vi "Task Loop.vi"(8 "error in (no error)":errorcluster, 11 "ChartGuiTask in":refnum<class "ChartGuiTask.lvclass">) -> (0 "error out":errorcluster)   [LabVIEW 2020, in "VolatusDemo.lvlib" / "ChartGuiTask.lvclass"]
uses:
  ChartGuiTask.lvclass
  C:/dev/lv20CE/relink/lv-volatus/Volatus/Task/Task.lvclass
  ChartGuiTask.lvclass/ChartGuiTask.ctl
  Volatus/Task/Task.lvclass/Task.ctl
  Volatus/Event API/EventAPI.lvclass/EventAPI.ctl
  Volatus/EventHandler Messages/Handle Event Msg/Handle Event Msg.lvclass/Handle Event Msg.ctl
  <vilib>/ActorFramework/Message Enqueuer/Message Enqueuer.lvclass/Message Enqueuer.ctl
  Volatus/Event API/Report Event.vi
  Volatus/EventHandler Messages/Handle Event Msg/Send Handle Event.vi
  <vilib>/ActorFramework/Message Enqueuer/Enqueue.vi
  Volatus/EventHandler Messages/Handle Event Msg/Handle Event Msg.lvclass
  C:/Program Files (x86)/National Instruments/LabVIEW 2020/vi.lib/ActorFramework/Message/Message.lvclass
  lv-vecto/Vecto/Group/Group.lvclass
  C:/dev/lv20CE/relink/lv-vecto/Vecto/GroupAbstract/GroupAbstract.lvclass
  <vilib>/ActorFramework/Message Priority Queue/Priority Enqueue.vi
  Volatus/Task/Task.lvclass
  lv-vecto/Vecto/GroupAbstract/GroupAbstract.lvclass
panel:
  out "Chart":dbl[][](graph)
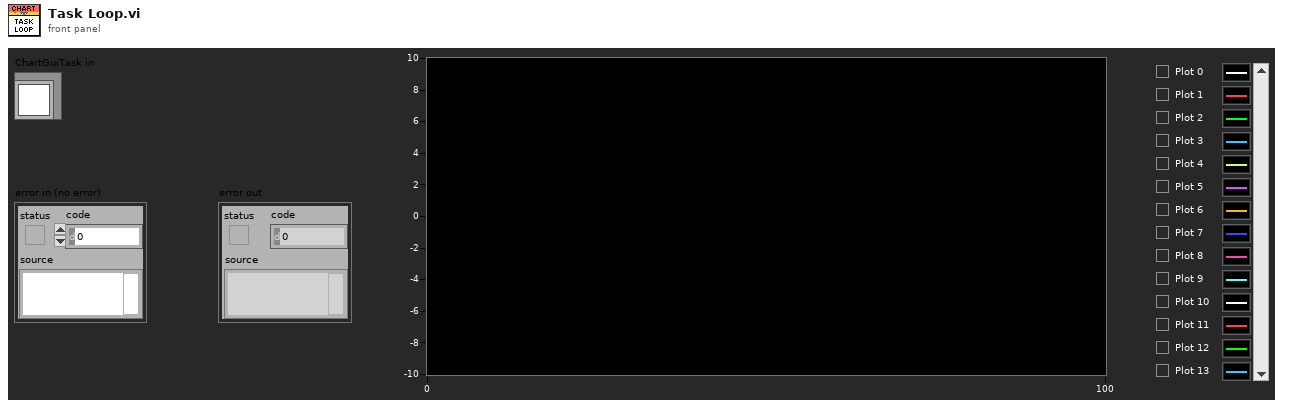
[diagram p1: front panel]
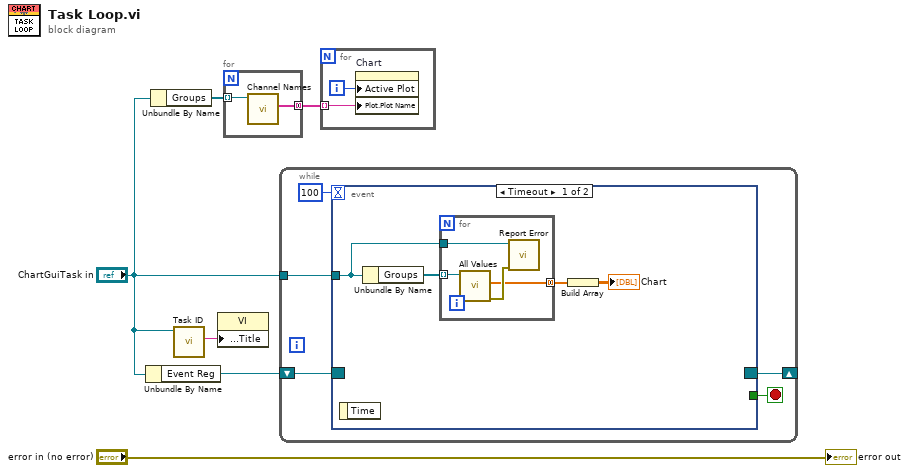
[diagram p0: block diagram]
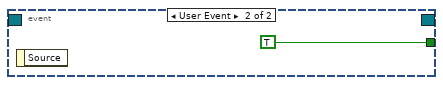
[diagram p2: hidden frame]
diagram:
  n1 = Unbundle By Name("ChartGuiTask in") -> ("Event Reg"=w5:refnum<event-registration>)
  n2 = Unbundle By Name("ChartGuiTask in") -> ("Groups"=w2:refnum<class "Group.lvclass">[])
  n3 = call-dynamic "Task ID.vi"("Task in"="ChartGuiTask in") -> ("Task ID"=w4:string)  [unwired: 8 in, 2 out]
  n4 = property class="VI"("Front Panel.Title"=w4) -> ()  [unwired: 2 in, 2 out]
  n5 = for {
    tunnel: w2 -> [w8] mode=indexing
    tunnel: [w7] -> w1 mode=concatenating
    n6 = call "Channel Names.vi"("GroupAbstract in"=w8) -> ("Channel Names"=w7:string[])  [unwired: 8 in, 2 out]
  }
  n7 = while {
    shift-right: [w11] -> _
    shift-left: w5 -> [w12]
    tunnel: "ChartGuiTask in" -> [w9]
    stop <- w10 stop-if-true
    n8 = event shown="[0] Timeout" {
      selector: w12 -> [_ _]
      dyn-events: [_ _] -> w11
      timeout: 100 -> [_ _]
      tunnel: [_ TRUE] -> w10
      tunnel: w9 -> [w14 _]
      event Timeout {
        n9 = event-data() -> ()  [unwired: 1 in, 1 out]
        n10 = Unbundle By Name(w14) -> ("Groups"=w15:refnum<class "Group.lvclass">[])
        n11 = for {
          tunnel: [w20] -> w17 mode=concatenating
          tunnel: w15 -> [w19] mode=indexing
          tunnel: w14 -> [w18]
          n12 = call "All Values.vi"("Group in"=w19) -> ("error out"=w21:errorcluster, "Scaled"=w20:dbl[])  [unwired: 6 in, 3 out]
          n13 = call "Report Error.vi"("error in (no error)"=w21, "Task in"=w18) -> ()  [unwired: 8 in, 2 out]
        }
        n14 = Build Array(w17) -> (→"Chart":dbl[][])
      }
      event User Event {
        n15 = event-data() -> ()  [unwired: 1 in, 1 out]
      }
    }
  }
  n16 = for {
    tunnel: w1 -> [w23] mode=indexing
    i -> [w24]
    n17 = property on="Chart" class="WFChart (strict)"("Active Plot"=w24, "Plot.Plot Name"=w23) -> ()  [unwired: 2 in, 2 out]
  }
  "error out" <- "error in (no error)"
